vi "display node data.vi"(8 "error in":errorcluster, 11 "NISE_CEF_serializable node in":refnum<class "NISE_CEF_serializable node.lvclass">) -> (0 "error out":errorcluster, 3 "NISE_CEF_serializable node out":refnum<class "NISE_CEF_serializable node.lvclass">)   [LabVIEW 2014, in "NISE_CEF_serializable node.lvclass"]
uses:
  NISE_CEF_serializable node.lvclass
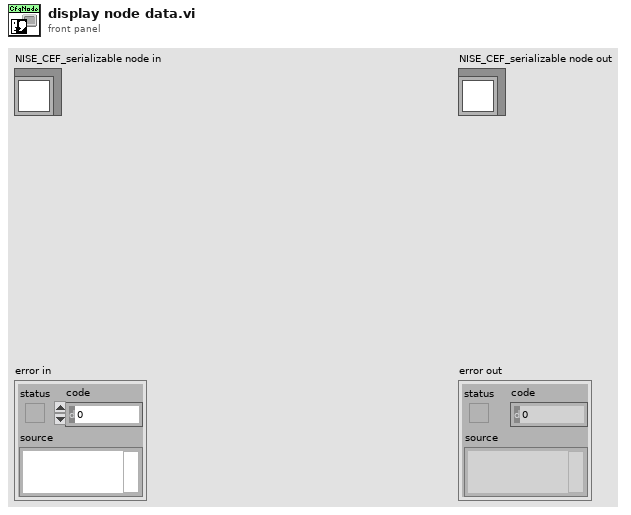
[diagram p1: front panel]
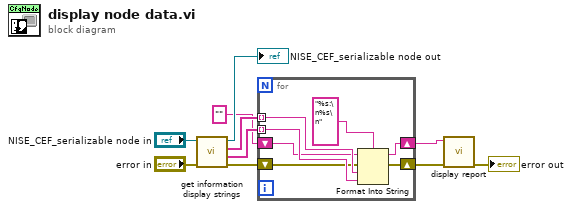
[diagram p0: block diagram]
diagram:
  n1 = call-dynamic "get information display strings.vi"("error in"="error in", "NISE_CEF_serializable node in"="NISE_CEF_serializable node in") -> ("error out"=w4:errorcluster, "Data"=w6:string[], "Labels"=w7:string[], "NISE_CEF_serializable node out"=→"NISE_CEF_serializable node out":refnum<class "NISE_CEF_serializable node.lvclass">)  [unwired: 6 in]
  n2 = for {
    tunnel: w7 -> [w17] mode=indexing
    tunnel: w6 -> [w16] mode=indexing
    shift-right: [w14] -> w1
    shift-left: "" -> [w13]
    shift-right: [w12] -> w3
    shift-left: w4 -> [w11]
    n3 = Format Into String(format string="%s:\n%s\n", initial string=w13, error in=w11, w17, w16) -> (resulting string=w14:string, error out=w12:errorcluster)
  }
  n4 = call "display report.vi"("error in"=w3, "data to display"=w1) -> ("error out"=→"error out":errorcluster)  [unwired: 9 in]
